vi "Handle Error.vi"(8 "error in (no error)":errorcluster, 11 "ZM-CM-communication_manager in":refnum<class "ZM-CM-communication_manager.lvclass">) -> (0 "error out":errorcluster, 2 "stop actor?":bool=TRUE, 3 "ZM-CM-communication_manager out":refnum<class "ZM-CM-communication_manager.lvclass">)   [LabVIEW 2020, in "ZM-CM-communication_manager.lvlib" / "ZM-CM-communication_manager.lvclass"]
doc: "Handle Error override of the communication manager: Call Parent first (it clears error 43 from a normal stop), then ZM-CM-evaluateError. Error-handling plan: none yet; evaluateError passes the error on, so an error stops the CM and, through its Last Ack, the root and the whole tree."
uses:
  ZM-CM-communication_manager.lvclass
  <vilib>/ActorFramework/Actor/Actor.lvclass
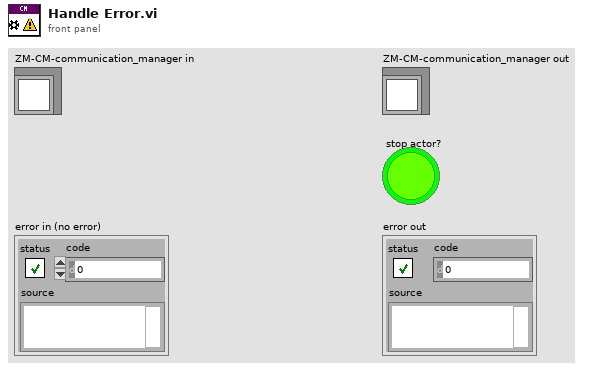
[diagram p1: front panel]
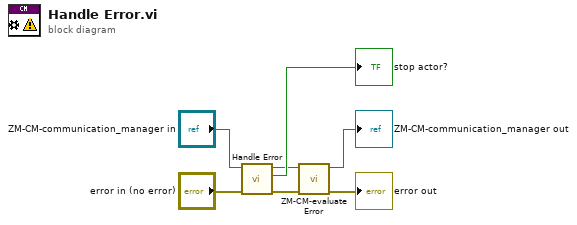
[diagram p0: block diagram]
diagram:
  n1 = call-parent "Handle Error.vi"("error in (no error)"="error in (no error)", "Actor in"="ZM-CM-communication_manager in") -> ("error out"=w1:errorcluster, "stop actor?"=→"stop actor?":bool, "Actor out"=w3:refnum<class "ZM-CM-communication_manager.lvclass">)  [unwired: 7 in]
  n2 = call "ZM-CM-evaluateError.vi"("error in (no error)"=w1, "ZM-CM-communication_manager in"=w3) -> ("error out"=→"error out":errorcluster, "ZM-CM-communication_manager out"=→"ZM-CM-communication_manager out":refnum<class "ZM-CM-communication_manager.lvclass">)  [unwired: 7 in, 1 out]
